vi "Initialization.vi"(8 "error in (no error)":errorcluster, 9 "UI Refs":T1, 10 "user event":T2, 11 "3way Lap in":refnum<class "3way Lap.lvclass">) -> (0 "error out":errorcluster, 3 "3way Lap out":refnum<class "3way Lap.lvclass">)   [LabVIEW 2025, in "Flow Grind.lvlib" / "3way Lap.lvclass"]
uses:
  3way Lap.lvclass
  C:/Users/Public/Documents/Sandia National Labs/TSS Plugin/Tests/XY Plotter.lvlibp/XY  Plotter/XY Plotter.lvclass
  Users/Public/Documents/Sandia National Labs/TSS Plugin/CEF.lvlibp/Node/UserEventRef.ctl
  Users/Public/Documents/Sandia National Labs/TSS Plugin/Tests/XY Plotter.lvlibp/XY Plotter configuration/XY Plotter configuration.lvclass
  Users/Public/Documents/Sandia National Labs/TSS Plugin/Tests/XY Plotter.lvlibp/XY Plotter configuration/Read XY Plotter.vi
  Users/Public/Documents/Sandia National Labs/TSS Plugin/Tests/XY Plotter.lvlibp/XY  Plotter/XY Plotter.lvclass
  Users/Public/Documents/Sandia National Labs/TSS Plugin/CEF.lvlibp/serializable configuration/CEF_serializable configuration.lvclass
  Users/Public/Documents/Sandia National Labs/TSS Plugin/CEF.lvlibp/Node/CEF_Node.lvclass
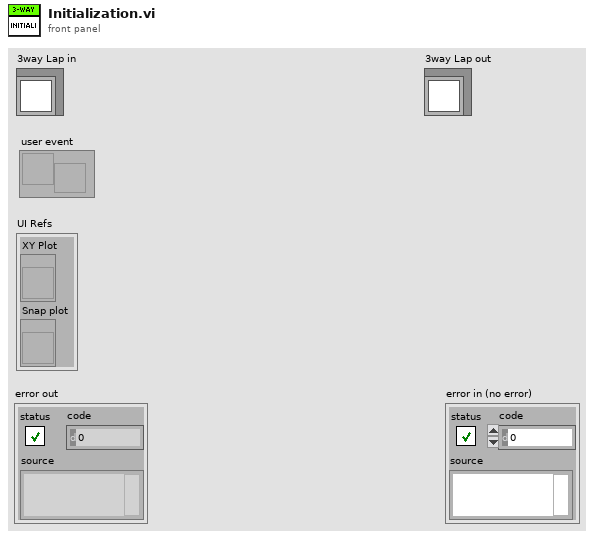
[diagram p1: front panel]
types:
  T1 = cluster{"XY Plot":refnum<vi>, "Snap plot":refnum<vi>}
  T2 = typedef "CEF.lvlibp/CEF_Node.lvclass/UserEventRef.ctl" = refnum<user-event>
  T3 = cluster{"Name":string, "Color":u32, "Style":u8, "Point Style":u8, "Name Visible":bool, "Allow Drag":bool, "Annotation Mode":u32, "Plot":i32, "Index":i32, "Position":cluster{"X":dbl, "Y":dbl}, "X Scale":u32, "Y Scale":u32, "Show Arrow":bool, "Lock Name":bool, "Plot Area":i32, "Label Offset":cluster{"X":dbl, "Y":dbl}}
  T4 = typedef "XY Plotter.lvlibp/XY Plotter configuration.lvclass/XY Plotter.ctl" = cluster{"Data Rate":i32, "Y-Scales":cluster{"Label":string, "Max":dbl, "Min":dbl, "Unit":enum16{"---", "V", "mA", "sec", "dB", "deg", "in/s", "in", "lbf", "Hz", "psi", "gpm"}, "Visible":bool}[], "Note":string, "History Length":i32, "DataLog Path":path, "Plot type":bool, "X-Scales":cluster{"Label":string, "Max":dbl, "Min":dbl, "Unit":enum16{"---", "V", "mA", "sec", "dB", "deg", "in/s", "in", "lbf", "Hz", "psi", "gpm"}, "Visible":bool}[], "Plot List":cluster{"Plot Name":string, "X Scale Index":u32, "Y Scale Index":u32, "Visible":bool}[]}
  T5 = cluster{"Label":string, "Max":dbl, "Min":dbl, "Unit":enum16{"---", "V", "mA", "sec", "dB", "deg", "in/s", "in", "lbf", "Hz", "psi", "gpm"}, "Visible":bool}[]
  T6 = cluster{"Plot Name":string, "X Scale Index":u32, "Y Scale Index":u32, "Visible":bool}[]
  T7 = cluster{"Label":string, "Max":dbl, "Min":dbl, "Unit":enum16{"---", "V", "mA", "sec", "dB", "deg", "in/s", "in", "lbf", "Hz", "psi", "gpm"}, "Visible":bool}
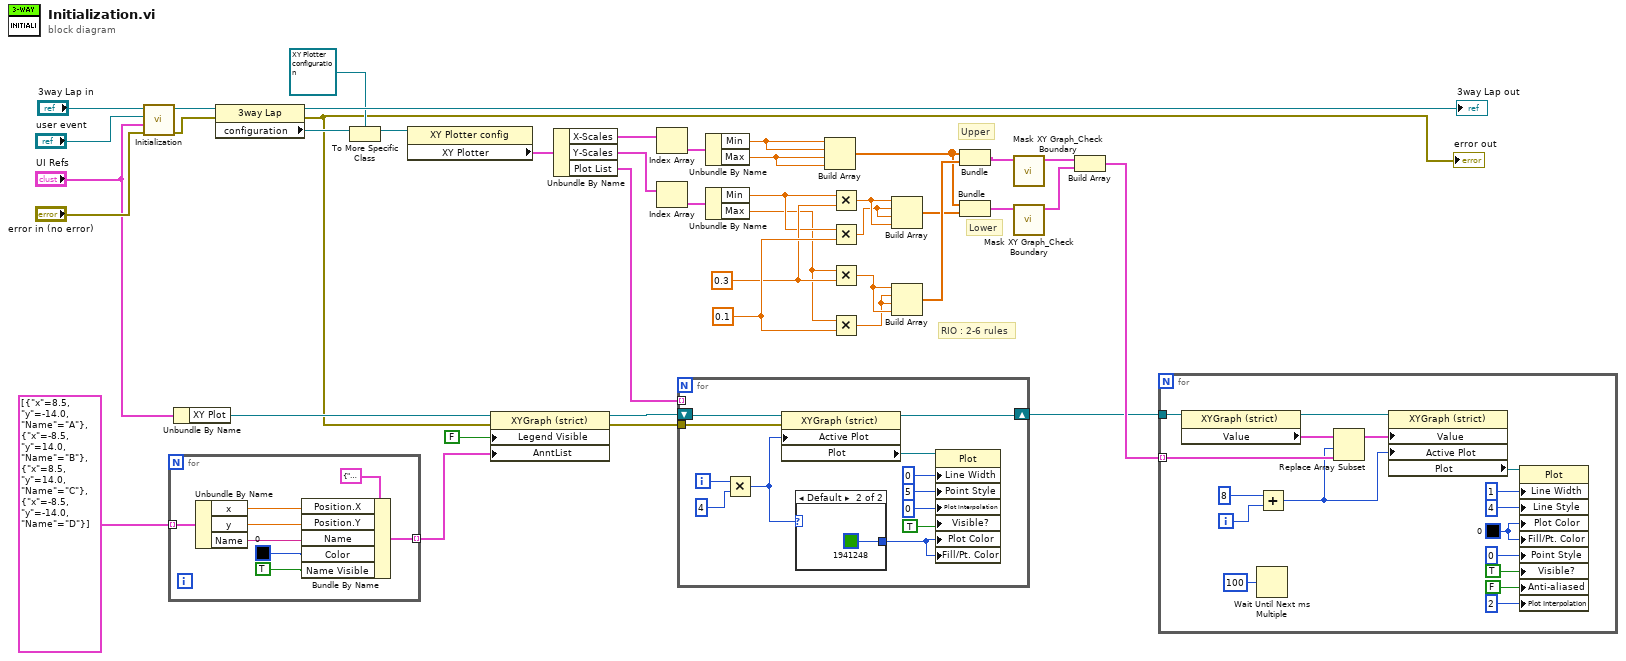
[diagram p0: block diagram]
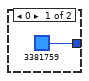
[diagram p2: hidden frame]
diagram:
  w12 = 0.1
  w11 = 0.3
  # "RIO : 2-6 rules"
  # "Lower"
  # "Upper"
  n1 = call-parent "Initialization.vi"("error in"="error in (no error)", "UI Refs"="UI Refs", "user event"="user event", "XY Plotter"="3way Lap in") -> ("error out"=w27:errorcluster, "XY Plotter out"=w39:refnum<class "3way Lap.lvclass">)  [unwired: 6 in]
  n2 = for {
    tunnel: cluster{"x":dbl, "y":dbl, "Name":string}[] [{"x"=8.5, "y"=-14.0, "Name"="A"}, {"x"=-8.5, "y"=14.0, "Name"="B"}, {"x"=8.5, "y"=14.0, "Name"="C"}, {"x"=-8.5, "y"=-14.0, "Name"="D"}] -> [w46] mode=indexing
    tunnel: [w47] -> w2 mode=indexing
    n3 = Unbundle By Name(w46) -> ("x"=w44:dbl, "y"=w43:dbl, "Name"=w45:string)
    n4 = Bundle By Name(cluster=T3 {"Name"="", "Color"=0, "Style"=0, "Point Style"=0, "Name Visible"=FALSE, "Allow Drag"=FALSE, "Annotation Mode"=0, "Plot"=0, "Index"=0, "Position"={"X"=0.0, "Y"=0.0}, "X Scale"=0, "Y Scale"=0, "Show Arrow"=FALSE, "Lock Name"=FALSE, "Plot Area"=0, "Label Offset"={"X"=0.0, "Y"=0.0}}, "Position.X"=w44, "Position.Y"=w43, "Name"=w45, "Color"=u32 0, "Name Visible"=TRUE) -> (w47:T3)
  }
  n5 = Unbundle By Name("UI Refs") -> ("XY Plot"=w24:refnum<vi>)
  n6 = property class="3way Lap"(reference=w39, error in=w27) -> (reference out=→"3way Lap out":refnum<class "3way Lap.lvclass">, error out=w1:errorcluster, "configuration"=w36:refnum<class "CEF_serializable configuration.lvclass">)
  "error out" <- w1
  n7 = To More Specific Class(target class=refnum<class "XY Plotter configuration.lvclass"> refnum ("XY Plotter.lvlibp:XY Plotter config"), reference=w36) -> (specific class reference=w35:refnum<class "XY Plotter configuration.lvclass">)  [unwired: 1 in, 1 out]
  n8 = property class="XY Plotter config"(reference=w35) -> ("XY Plotter"=w33:T4)  [unwired: 1 in, 2 out]
  n9 = property class="XYGraph (strict)"(reference=w24, error in=w1, "Legend Visible"=FALSE ("Cursor Legend Visible"), "AnntList"=w2) -> (reference out=w23:refnum<vi>, error out=w25:errorcluster)
  n10 = Unbundle By Name(w33) -> ("X-Scales"=w21:T5, "Y-Scales"=w20:T5, "Plot List"=w26:T6)
  n11 = Index Array(array=w21) -> (element=w10:T7)  [unwired: 1 in]
  n12 = Index Array(array=w20) -> (element=w9:T7)  [unwired: 1 in]
  n13 = for {
    shift-right: [w61] -> w4
    shift-left: w23 -> [w62]
    tunnel: w26 -> [_] mode=indexing
    tunnel: w25 -> [w56]
    i -> [w54]
    n14 = Multiply(x=w54, y=4) -> (x*y=w52:i32)
    n15 = property class="XYGraph (strict)"(reference=w62, error in=w56, "Active Plot"=w52) -> (reference out=w61:refnum<vi>, "Plot"=w57:refnum<vi>)  [unwired: 1 out]
    n16 = case shown="Default" w52 {
      tunnel: [u32 3381759 ("Plot Color") u32 1941248 ("Plot Color")] -> w51
      frame 0 {
      }
      frame Default {
      }
    }
    n17 = property class="Plot"(reference=w57, "Line Width"=u8 0, "Point Style"=u8 5, "Plot Interpolation"=u8 0, "Visible?"=TRUE ("Visible"), "Plot Color"=w51, "Fill/Pt. Color"=w51) -> ()  [unwired: 1 in, 2 out]
  }
  n18 = Unbundle By Name(w10) -> ("Min"=w8:dbl, "Max"=w7:dbl)
  n19 = Unbundle By Name(w9) -> ("Min"=w6:dbl, "Max"=w5:dbl)
  n20 = Build Array(w8, w8, w7, w7) -> (w16:dbl[])
  n21 = Multiply(x=w6, y=w11) -> (x*y=w15:dbl)
  n22 = Multiply(x=w6, y=w12) -> (x*y=w14:dbl)
  n23 = Multiply(x=w5, y=w11) -> (x*y=w19:dbl)
  n24 = Multiply(x=w5, y=w12) -> (x*y=w18:dbl)
  n25 = Build Array(w15, w14, w14, w15) -> (w13:dbl[])
  n26 = Build Array(w19, w18, w18, w19) -> (w17:dbl[])
  n27 = Bundle(w16, w17) -> (w31:cluster{dbl[], dbl[]})  [unwired: 1 in]
  n28 = Bundle(w16, w13) -> (w32:cluster{dbl[], dbl[]})  [unwired: 1 in]
  n29 = call "Mask XY Graph_Check Boundary.vi"("Boundary"=w31) -> ("Closed Boundary"=w29:cluster{"X":dbl[], "Y":dbl[]})  [unwired: 9 in, 1 out]
  n30 = call "Mask XY Graph_Check Boundary.vi"("Boundary"=w32) -> ("Closed Boundary"=w28:cluster{"X":dbl[], "Y":dbl[]})  [unwired: 9 in, 1 out]
  n31 = Build Array(w29, w28) -> (w30:cluster{"X":dbl[], "Y":dbl[]}[])
  n32 = for {
    tunnel: w30 -> [w77] mode=indexing
    tunnel: w4 -> [w78]
    i -> [w76]
    w65 = u32 0 ("Plot Color")
    n33 = property class="XYGraph (strict)"(reference=w78) -> (reference out=w79:refnum<vi>, "Value"=w80:cluster{dbl[], dbl[]}[])  [unwired: 1 in, 1 out]
    n34 = Wait Until Next ms Multiple(millisecond multiple=u32 100) -> ()  [unwired: 1 out]
    n35 = Add(x=8, y=w76) -> (x+y=w73:i32)
    n36 = Replace Array Subset(array=w80, new element=w77, index=w73) -> (w81:cluster{dbl[], dbl[]}[])
    n37 = property class="XYGraph (strict)"(reference=w79, "Value"=w81, "Active Plot"=w73) -> ("Plot"=w66:refnum<vi>)  [unwired: 1 in, 2 out]
    n38 = property class="Plot"(reference=w66, "Line Width"=u8 1, "Line Style"=u8 4, "Plot Color"=w65, "Fill/Pt. Color"=w65, "Point Style"=u8 0, "Visible?"=TRUE ("Visible"), "Anti-aliased"=FALSE, "Plot Interpolation"=u8 2) -> ()  [unwired: 1 in, 2 out]
  }
